vi "Build Data Frame.vi"(0 "RFFE RegWrite Command in":refnum<class "RFFE RegWrite Command.lvclass">, 11 "error in (no error)":errorcluster) -> (4 "RFFE RegWrite Command out":refnum<class "RFFE RegWrite Command.lvclass">, 6 "Data Frame":u8[](array[numeric]), 15 "error out":errorcluster)   [LabVIEW 2018, in "MIPI RFFE API.lvlib" / "RFFE RegWrite Command.lvclass"]
uses:
  RFFE RegWrite Command.lvclass
  C:/Users/semoore/Projects/mipi-rffe-labview-oop/Standard Command/RFFE Standard Command.lvclass
  Standard Command/RFFE Standard Command.lvclass/RFFE Standard Command.ctl
  Standard Command/Get Register Data.vi
  MIPI RFFE API.lvlib
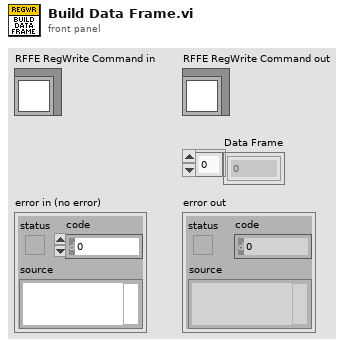
[diagram p1: front panel]
types:
  T1 = typedef "RFFE Commands.lvlib/Register Data.ctl" = u8
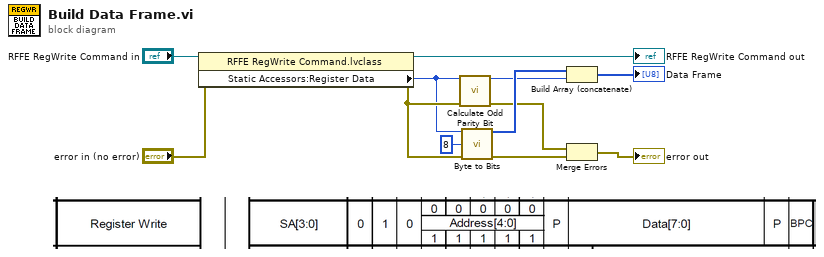
[diagram p0: block diagram]
diagram:
  n1 = property class="RFFE RegWrite Command.lvclass"(reference="RFFE RegWrite Command in", error in="error in (no error)") -> (reference out=→"RFFE RegWrite Command out":refnum<class "RFFE RegWrite Command.lvclass">, error out=w2:errorcluster, "Static Accessors:Register Data"=w1:T1)
  n2 = call "Calculate Odd Parity Bit.vi"("Byte"=w1, "error in (no error)"=w2) -> ("Odd Parity Bit"=w5:u8, "error out"=w4:errorcluster)  [unwired: 12 in]
  n3 = call "Byte to Bits.vi"("Byte"=w1, "Bit Width"=8, "error in (no error)"=w2) -> ("Bits"=w6:u8[], "error out"=w3:errorcluster)  [unwired: 11 in]
  n4 = Build Array (concatenate)(w6, w5) -> (→"Data Frame":u8[])
  n5 = Merge Errors(w4, w3) -> (→"error out":errorcluster)
